vi "Configure Module.vi"(8 "error in (no error)":errorcluster, 10 "IOV ref in":variant, 11 "Module Template in":refnum<class "9234.lvclass">) -> (0 "error out":errorcluster, 2 "IOV ref out":variant, 3 "Module Template out":refnum<class "9234.lvclass">)   [LabVIEW 2020, in "Modules.lvlib" / "9234.lvclass"]
uses:
  9234.lvclass
  <resource>/objmgr/cRIO.rc
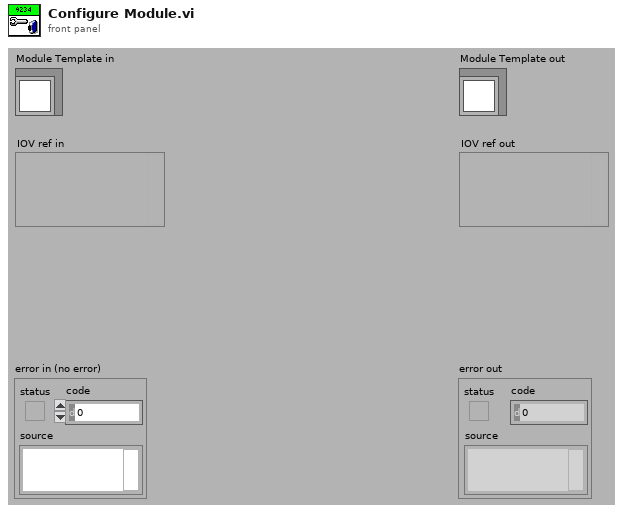
[diagram p1: front panel]
types:
  T1 = typedef "Modules.lvlib/9234.lvclass/Data rate.ctl" = u32
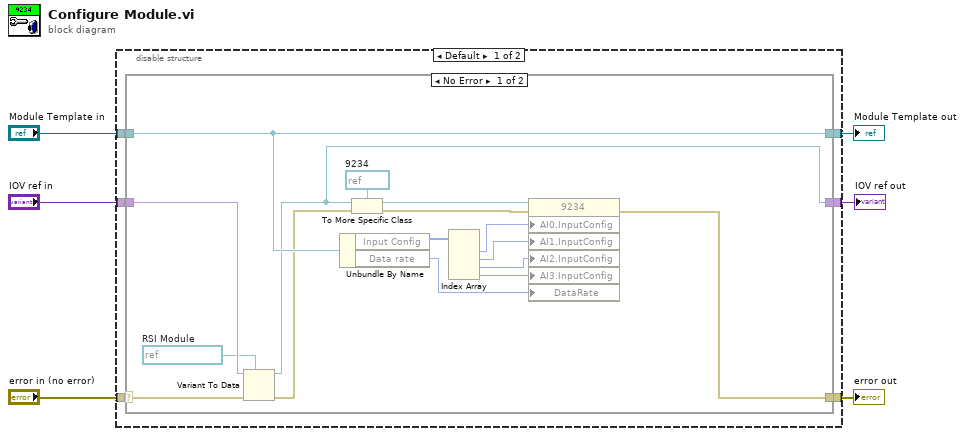
[diagram p0: block diagram]
diagram:
  n1 = disable-structure shown="Default" {
    disable-tunnel: "error in (no error)" -> [w12 w32]
    disable-tunnel: [w11 w32] -> w5
    disable-tunnel: "Module Template in" -> [w10 w34]
    disable-tunnel: [w9 w34] -> w3
    disable-tunnel: "IOV ref in" -> [w8 w33]
    disable-tunnel: [w7 w33] -> w1
    frame condition #0 {
      n2 = case shown="No Error" w12 {
        selector: w12 -> [w27 w31]
        tunnel: [w23 w31] -> w11
        tunnel: [w28 w30] -> w9
        tunnel: w10 -> [w28 w30]
        tunnel: w8 -> [w15 w29]
        tunnel: [w14 w29] -> w7
        frame No Error {
          w13 = refnum<k21> refnum  # RSI Module
          w26 = refnum<k21> refnum  # 9234
          n3 = Variant To Data(error in=w27, type=w13, Variant=w15) -> (data=w14:refnum<k21>, error out=w16:errorcluster)
          n4 = Unbundle By Name(w28) -> ("Input Config"=w22:u32[], "Data rate"=w17:T1)
          n5 = To More Specific Class(target class=w26, reference=w14, error in=w16) -> (specific class reference=w25:refnum<k21>, error out=w24:errorcluster)
          n6 = Index Array(array=w22) -> (element #1=w21:u32, element #2=w20:u32, element #3=w19:u32, element #4=w18:u32)  [unwired: 4 in]
          n7 = property class="9234"(reference=w25, error in=w24, "AI0.InputConfig"=w21, "AI1.InputConfig"=w20, "AI2.InputConfig"=w19, "AI3.InputConfig"=w18, "DataRate"=w17) -> (error out=w23:errorcluster)  [unwired: 1 out]
        }
        frame Error {
        }
      }
    }
    frame condition #1 (active) {
    }
  }
  "error out" <- w5
  "Module Template out" <- w3
  "IOV ref out" <- w1
